vi "Tester - Append to Circular Buffer.vi"() -> ()   [LabVIEW 2026, in "RSysUtils Array.lvlib"]
uses:
  RSysUtils Array.lvlib
  2b3b347f-d5d1-46c7-b56b-93d962828585.vi
panel:
  out "Circular Buffer":i32[](array[numeric])
  out "Was Oldest Element Removed?":bool
  out "Was New Element Added?":bool
  in  "Max No. of Elements":u32=10
  in  "New Element":i32=147
  in  "Append to Circular Buffer":bool
  out "Loop iteration":i32
  in  "Stop":bool
  # "Tester\nAppend to Circular Buffer.vim"
  # "Inputs"
  # "Outputs"
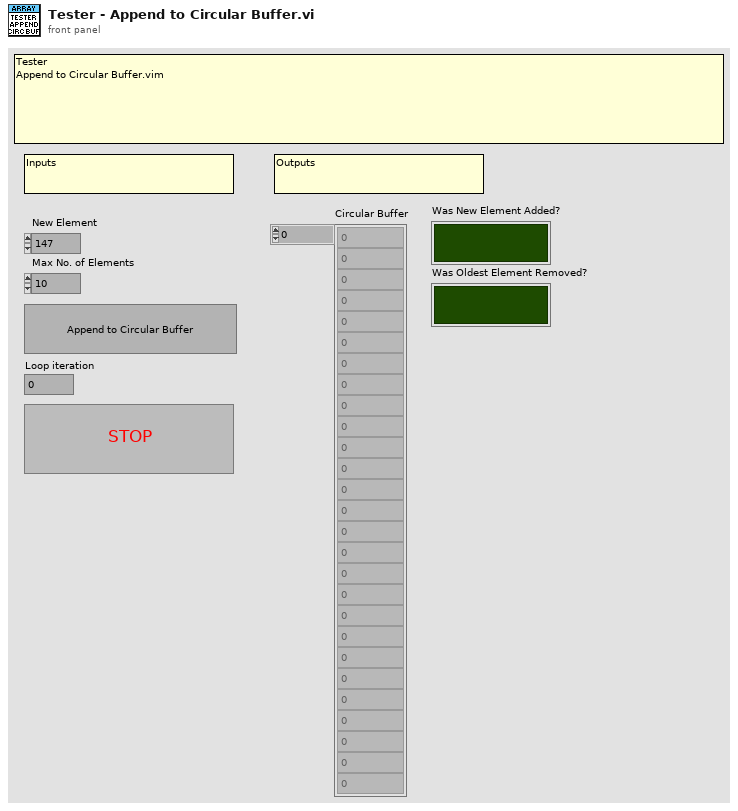
[diagram p1: front panel]
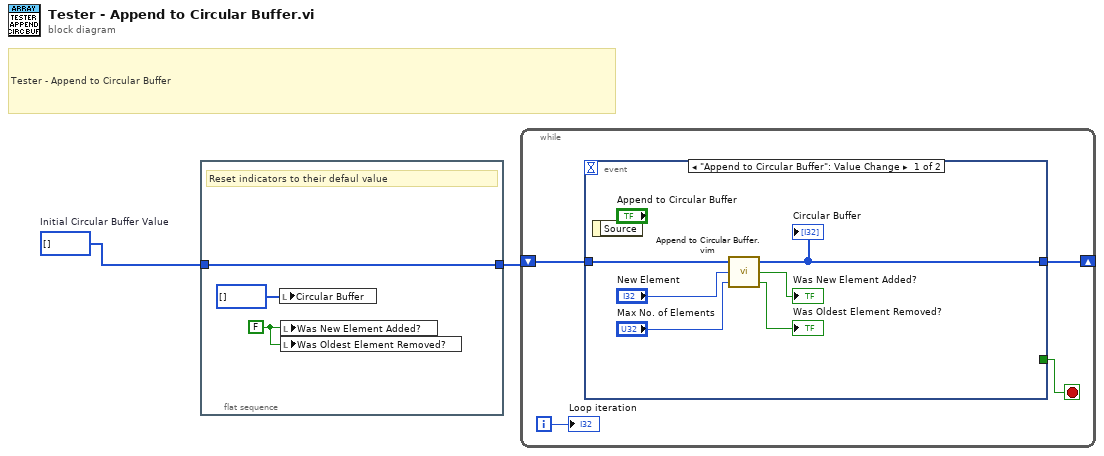
[diagram p0: block diagram]
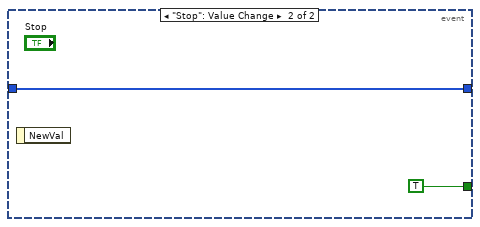
[diagram p2: hidden frame]
diagram:
  w1 = i32[] []  # Initial Circular Buffer Value
  # "Tester - Append to Circular Buffer"
  n1 = flat-sequence {
    tunnel: [w5] -> w2
    tunnel: w1 -> [w5]
    frame #0 {
      w3 = FALSE
      # "Reset indicators to their defaul value"
      n2 = local write "Circular Buffer"(i32[] [] ("Circular Buffer")) -> ()
      n3 = local write "Was New Element Added?"(w3) -> ()
      n4 = local write "Was Oldest Element Removed?"(w3) -> ()
    }
  }
  n5 = while {
    shift-right: [w6] -> _
    shift-left: w2 -> [w7]
    i -> [w8]
    stop <- w9 stop-if-true
    n6 = event shown="[0] \"Append to Circular Buffer\": Value Change" {
      selector: _ -> [_ _]
      dyn-events: _ -> [_ _]
      timeout: _ -> [_ _]
      tunnel: [_ TRUE] -> w9
      tunnel: w7 -> [w15 w16]
      tunnel: [w14 w16] -> w6
      event "Append to Circular Buffer": Value Change {
        n7 = event-data() -> ()  [unwired: 1 in, 1 out]
        n8 = call "Append to Circular Buffer.vim"("Max No. of Elements"="Max No. of Elements", "New Element"="New Element", "Circular Buffer In"=w15) -> ("Was Oldest Element Removed?"=→"Was Oldest Element Removed?":bool, "Was New Element Added?"=→"Was New Element Added?":bool, "Circular Buffer Out"=w14:i32[])
        "Circular Buffer" <- w14
      }
      event "Stop": Value Change {
        n9 = event-data() -> ()  [unwired: 1 in, 1 out]
      }
    }
    "Loop iteration" <- w8
  }
